vi "Choix visu b.vi"(3 "Noms":string[](array[string])=["un", "deux", "trois", "quatre", "cinq", "six", "sept", "huit", "neuf", "dix", "onze", "douze"]) -> (0 "annulé":bool, 1 "Noms 2":string[](array[string])=["un", "deux", "trois", "quatre", "cinq", "six", "sept", "huit", "neuf", "dix", "onze", "douze"])   [LabVIEW 2022 SP3]
uses:
  Variables globales/Variable glob generale.vi
panel:
  in  "annuler":bool
  in  "OK":bool
  in  "choisir les capteurs à visualiser :":i32[](listbox)
  # "limiter la visualisation\nà certains capteurs\n(l'enregistrement continue sur l'ensemble des capteurs)"
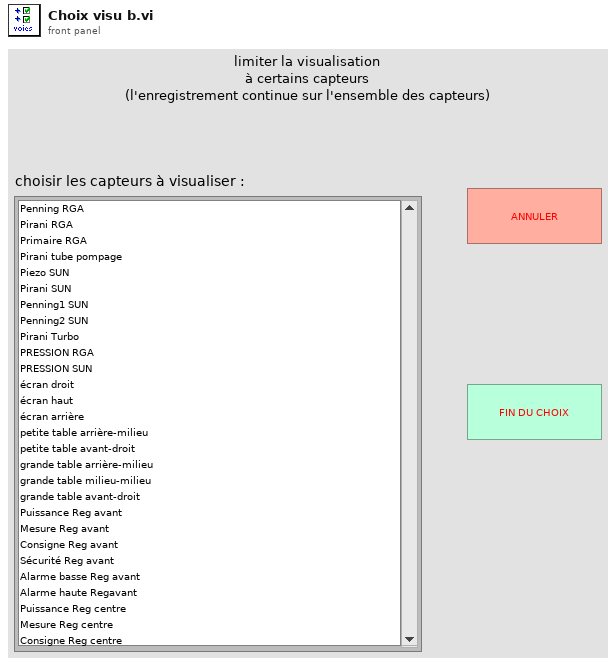
[diagram p1: front panel]
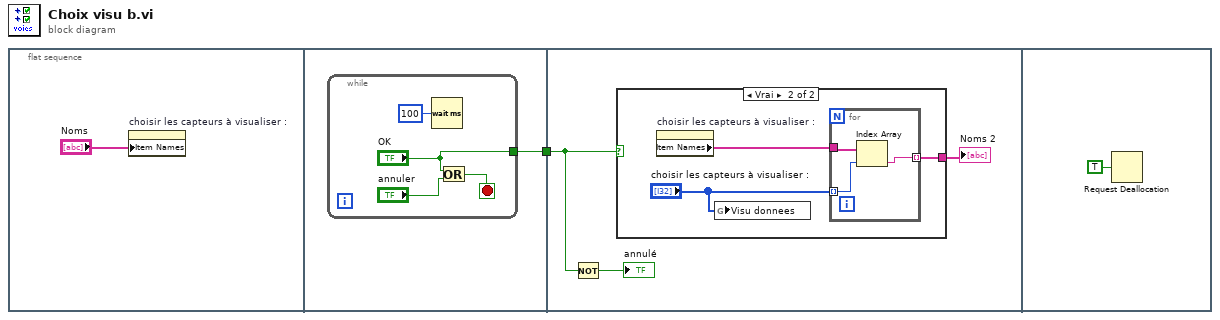
[diagram p0: block diagram]
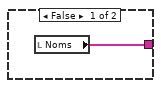
[diagram p2: hidden frame]
diagram:
  n1 = flat-sequence {
    tunnel: [w3] -> w1
    tunnel: w1 -> [w10]
    frame #0 {
      n2 = property on="choisir les capteurs à visualiser :" class="LstDér (strict)"("Item Names"="Noms") -> ()  [unwired: 2 in, 2 out]
    }
    frame #1 {
      n3 = while {
        tunnel: ["OK"] -> w3
        stop <- w5 stop-if-true
        n4 = Wait (ms)(milliseconds to wait=u32 100 ("attente (ms)")) -> ()  [unwired: 1 out]
        n5 = Or(x="OK", y="annuler") -> (x .or. y?=w5:bool)
      }
    }
    frame #2 {
      n6 = Not(x=w10) -> (.not. x?=→"annulé":bool)
      n7 = case shown="Vrai" w10 {
        tunnel: [w11 w13] -> w9
        frame False {
          n8 = local read "Noms"() -> (w11:string[])
        }
        frame True {
          n9 = property on="choisir les capteurs à visualiser :" class="LstDér (strict)"() -> ("Item Names"=w14:string[])  [unwired: 2 in, 2 out]
          n10 = global write "Variable glob generale.vi" "Visu donnees"("choisir les capteurs à visualiser :") -> ()
          n11 = for {
            tunnel: "choisir les capteurs à visualiser :" -> [w16] mode=indexing
            tunnel: w14 -> [w17]
            tunnel: [w15] -> w13 mode=indexing
            n12 = Index Array(array=w17, index=w16) -> (element=w15:string)
          }
        }
      }
      "Noms 2" <- w9
    }
    frame #3 {
      n13 = Request Deallocation(TRUE ("flag")) -> ()
    }
  }
